vi "VIH HelpGen - HTML - Read HTML Title.vi"(8 "error in":errorcluster, 11 "HTML File Path":path) -> (0 "error out":errorcluster, 2 "Title":string, 3 "dup HTML File Path":path)   [LabVIEW 2014]
doc: "::: VI Helpeks :::\nCopyright (c) 2000-2026 Konstantin Shifershteyn. All rights reserved."
panel:
  # "VI Helpeks\nCopyright (c) 2012-2026 Konstantin Shifershteyn"
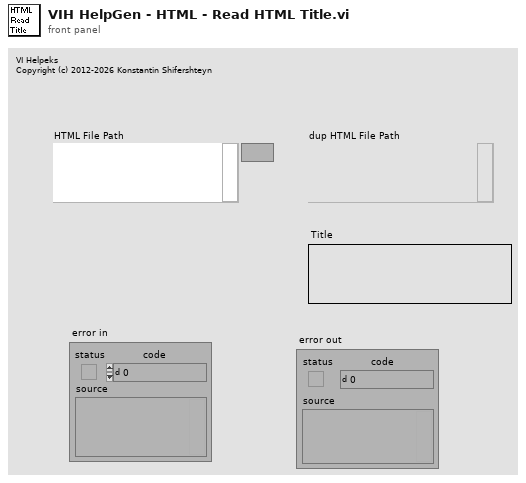
[diagram p1: front panel]
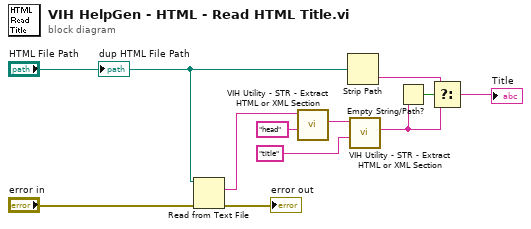
[diagram p0: block diagram]
diagram:
  n1 = Read from Text File(file (use dialog)="HTML File Path", error in="error in") -> (text=w5:string, error out=→"error out":errorcluster)  [unwired: 2 in, 2 out]
  n2 = call "VIH Utility - STR - Extract HTML or XML Section.vi"("Section name"="head", "HTML in"=w5) -> ("body"=w7:string)  [unwired: 5 in, 4 out]
  n3 = Strip Path(path="HTML File Path") -> (name=w11:string)  [unwired: 1 out]
  n4 = call "VIH Utility - STR - Extract HTML or XML Section.vi"("Section name"="title", "HTML in"=w7) -> ("body"=w9:string)  [unwired: 5 in, 4 out]
  n5 = Empty String/Path?(string/path=w9) -> (empty?=w10:bool)
  n6 = Select(t=w11, s=w10, f=w9) -> (s? t:f=→"Title":string)
  "dup HTML File Path" <- "HTML File Path"
